vi "VIH Utility - APP - State Queue Parser (STR).vi"(9 "input queue":string) -> (0 "state parameters":string, 2 "state":string, 3 "remained queue":string, 4 "complete state specifier":string)   [LabVIEW 2014]
doc: "::: VI Helpeks :::\nCopyright (c) 2000-2026 Konstantin Shifershteyn. All rights reserved."
panel:
  # "VI Helpeks\nCopyright (c) 2012-2026 Konstantin Shifershteyn"
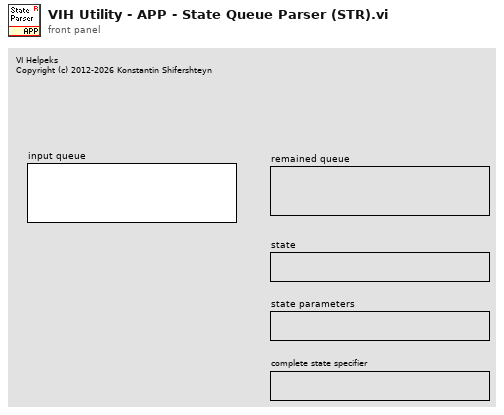
[diagram p1: front panel]
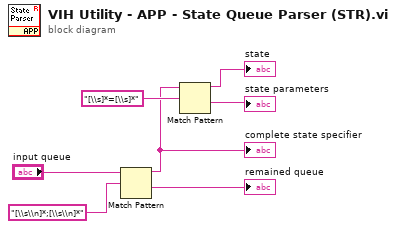
[diagram p0: block diagram]
diagram:
  n1 = Match Pattern(string="input queue", regular expression="[\\s\\n]*;[\\s\\n]*") -> (before substring=w6:string, after substring=→"remained queue":string)  [unwired: 3 out]
  "complete state specifier" <- w6
  n2 = Match Pattern(string=w6, regular expression="[\\s]*=[\\s]*") -> (before substring=→"state":string, after substring=→"state parameters":string)  [unwired: 3 out]
